vi "1m back.vi"   [LabVIEW 2017]
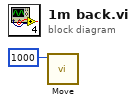
[diagram p0: block diagram]
diagram:
  n1 = call "Move.vi"("Distance (mm)"=1000) -> ()  [unwired: 9 in]
